vi "JSON item equals.vi"(8 "error in (no error)":errorcluster, 9 "expected":string, 10 "path":string, 11 "JSON":string) -> (0 "error out":errorcluster, 2 "item":string, 3 "equal?":bool)   [LabVIEW 2020, in "MCP Server tests.lvlib"]
doc: "Test helper. Looks up path in JSON and compares the item's raw JSON text with expected, so a string is expected with its quotes and a number as written.\n\nA missing item gives equal? FALSE and the lookup error in error out."
uses:
  MCP Server tests.lvlib
  <vilib>/JDP Science/JSONtext/Next JSON Value.vi
  <vilib>/JDP Science/JSONtext/String Subset.vi
  <vilib>/JDP Science/JSONtext/Parsing/Advance past next JSON Value (inlined COPY).vi
  <vilib>/JDP Science/JSONtext/Parsing/Advance past whitespace.vi
  <vilib>/JDP Science/JSONtext/Parsing/Advance past String.vi
  <vilib>/JDP Science/JSONtext/Parsing/Advance past Number.vi
  <vilib>/JDP Science/JSONtext/Parsing/Advance past Line Ending.vi
  <vilib>/JDP Science/JSONtext/Parsing/Parse Full Path or Item Name.vi
  <vilib>/JDP Science/JSONtext/Parsing/Advance past Array.vi
  <vilib>/JDP Science/JSONtext/Parsing/Advance past Object.vi
  <vilib>/JDP Science/JSONtext/support/Error Cluster From Code.vi
  <vilib>/JDP Science/JSONtext/Offset/Find Item Locations by Path.vi
  <vilib>/JDP Science/JSONtext/JSONtext.lvlib
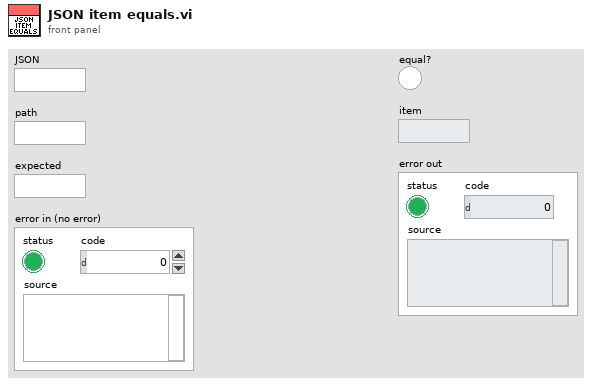
[diagram p1: front panel]
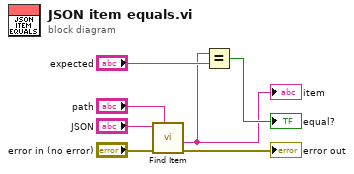
[diagram p0: block diagram]
diagram:
  n1 = call <vilib>:"Find Item.vi"("$Path or Item Name"="path", "error in (no error)"="error in (no error)", "JSON"="JSON") -> ("error out"=→"error out":errorcluster, "<JSON>"=w2:string)  [unwired: 5 in, 2 out]
  "item" <- w2
  n2 = Equal?(x=w2, y="expected") -> (x = y?=→"equal?":bool)
